vi "Get Master and Local Mod IOVs.vi"(6 "Disable Refresh Modules":bool, 8 "error in (no error)":errorcluster, 11 "IOV Engine in":refnum<k21>="ni.var.io:/") -> (0 "error IO":errorcluster, 1 "All Masters":refnum<k21>[](array[refnum]), 2 "All Local Mods":refnum<k21>[](array[refnum]), 3 "Local UDV Container":refnum<k21>[](array[refnum]))   [LabVIEW 2020, in "SEECD Engine.lvlib"]
uses:
  SEECD Engine.lvlib
  <resource>/objmgr/ni.var.rc
  <vilib>/NI VeriStand/Custom Device Tools/Custom Device Utility Library/Custom Device Utility Library.lvlib
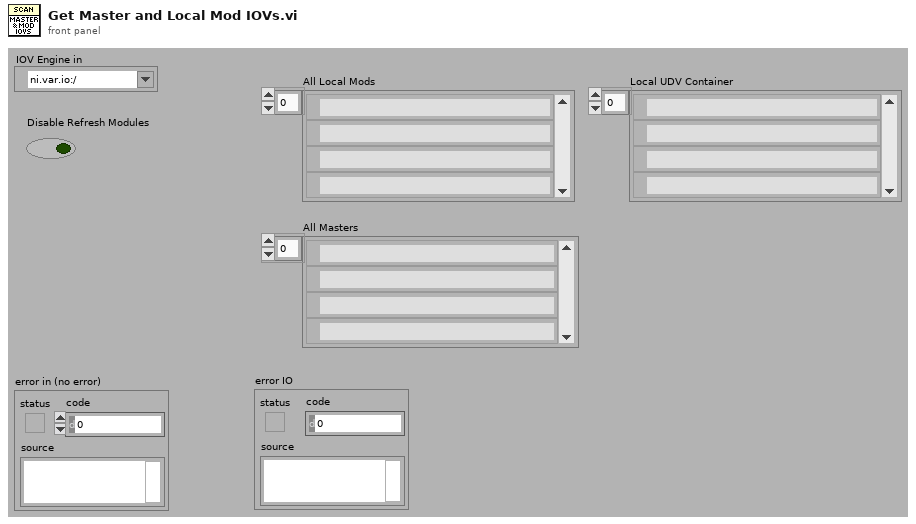
[diagram p1: front panel]
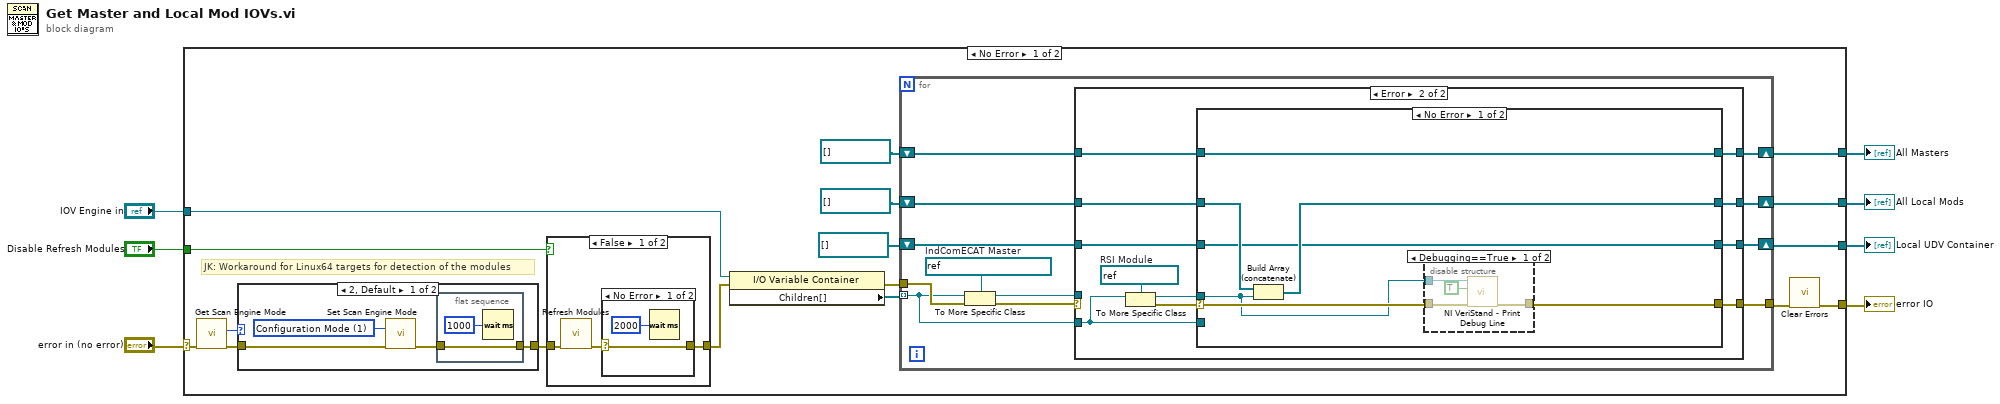
[diagram p0: block diagram]
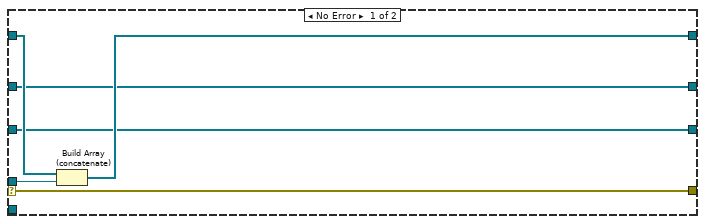
[diagram p5: hidden frame]
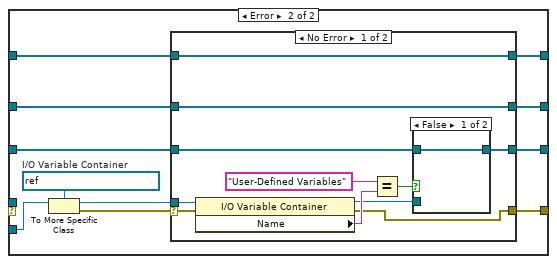
[diagram p7: hidden frame]
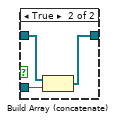
[diagram p8: hidden frame]
diagram:
  n1 = case shown="No Error" "error in (no error)" {
    selector: "error in (no error)" -> [w11 w110]
    tunnel: [w24 w110] -> w7
    tunnel: [w21 _] -> w6
    tunnel: "IOV Engine in" -> [w18 _]
    tunnel: [w16 _] -> w3
    tunnel: [w14 _] -> w2
    tunnel: "Disable Refresh Modules" -> [w8 _]
    frame No Error {
      # "JK: Workaround for Linux64 targets for detection of the modules"
      n2 = call <vilib>:"Get Scan Engine Mode.vi"("error in (no error)"=w11) -> ("error out"=w13:errorcluster, "mode"=w12:i32)  [unwired: 9 in]
      n3 = case shown="2, Default" w12 {
        tunnel: w13 -> [w34 w38]
        tunnel: [w33 w38] -> w9
        frame 2, Default {
          w35 = 1 items=["Configuration Mode"=1, "Active Mode"=2] ("mode (Active Mode)")
          n4 = call <vilib>:"Set Scan Engine Mode.vi"("mode (Active Mode)"=w35, "error in (no error)"=w34) -> ("error out"=w32:errorcluster)  [unwired: 13 in]
          n5 = flat-sequence {
            tunnel: [w37] -> w33
            tunnel: w32 -> [w37]
            frame #0 {
              n6 = Wait (ms)(milliseconds to wait=u32 1000) -> ()  [unwired: 1 out]
            }
          }
        }
        frame 1 {
        }
      }
      n7 = case shown="False" w8 {
        tunnel: [w26 w31] -> w10
        tunnel: w9 -> [w25 w31]
        frame False {
          n8 = call <vilib>:"Refresh Modules.vi"("error in (no error)"=w25) -> ("error out"=w27:errorcluster)  [unwired: 10 in]
          n9 = case shown="No Error" w27 {
            selector: w27 -> [w28 w30]
            tunnel: [w28 w30] -> w26
            frame No Error {
              n10 = Wait (ms)(milliseconds to wait=u32 2000) -> ()  [unwired: 1 out]
            }
            frame Error {
            }
          }
        }
        frame True {
        }
      }
      n11 = property class="I/O Variable Container"(reference=w18, error in=w10) -> (error out=w20:errorcluster, "Children[]"=w19:refnum<k21>[])  [unwired: 1 out]
      n12 = for {
        tunnel: w19 -> [w43] mode=indexing
        tunnel: w20 -> [w50]
        shift-right: [w46] -> w21
        shift-left: refnum<k21>[] [] -> [w45]
        tunnel: [w44] -> w23
        shift-right: [w41] -> w16
        shift-left: refnum<k21>[] [] -> [w42]
        shift-right: [w39] -> w14
        shift-left: refnum<k21>[] [] -> [w40]
        w49 = refnum<k21> refnum  # IndComECAT Master
        n13 = To More Specific Class(target class=w49, reference=w43, error in=w50) -> (specific class reference=w47:refnum<k21>, error out=w48:errorcluster)
        n14 = case shown="Error" w48 {
          selector: w48 -> [w54 _]
          tunnel: w47 -> [w51 _]
          tunnel: [w56 w61] -> w46
          tunnel: w45 -> [w55 w62]
          tunnel: [w54 w60] -> w44
          tunnel: w43 -> [_ w59]
          tunnel: w42 -> [w53 w64]
          tunnel: [w53 w63] -> w41
          tunnel: w40 -> [w52 w58]
          tunnel: [w52 w57] -> w39
          frame No Error {
            n15 = Build Array (concatenate)(w55, w51) -> (w56:refnum<k21>[])
          }
          frame Error {
            w67 = refnum<k21> refnum  # RSI Module
            n16 = To More Specific Class(target class=w67, reference=w59) -> (specific class reference=w65:refnum<k21>, error out=w66:errorcluster)  [unwired: 1 in]
            n17 = case shown="No Error" w66 {
              tunnel: w65 -> [w68 _]
              selector: w66 -> [w69 _]
              tunnel: w64 -> [w74 w86]
              tunnel: [w73 w83] -> w63
              tunnel: w62 -> [w72 w85]
              tunnel: [w72 w84] -> w61
              tunnel: [w70 w80] -> w60
              tunnel: w59 -> [_ w89]
              tunnel: w58 -> [w71 w87]
              tunnel: [w71 w82] -> w57
              frame No Error {
                n18 = Build Array (concatenate)(w74, w68) -> (w73:refnum<k21>[])
                n19 = disable-structure shown="Debugging==True" {
                  disable-tunnel: [w78 w79] -> w70
                  disable-tunnel: w69 -> [w77 w79]
                  disable-tunnel: w68 -> [w76 _]
                  frame condition #0 {
                    n20 = call <vilib>:"NI VeriStand - Print Debug Line.vi"("error in (no error)"=w77, "Add to log file? (F)"=TRUE, "Message"=w76) -> ("error out"=w78:errorcluster)  [unwired: 8 in]
                  }
                  frame condition #1 (active) {
                  }
                }
              }
              frame Error {
                w90 = refnum<k21> refnum  # I/O Variable Container
                n21 = To More Specific Class(target class=w90, reference=w89) -> (specific class reference=w81:refnum<k21>, error out=w88:errorcluster)  [unwired: 1 in]
                n22 = case shown="No Error" w88 {
                  selector: w88 -> [w99 w106]
                  tunnel: w87 -> [w93 w109]
                  tunnel: w86 -> [w100 w108]
                  tunnel: w85 -> [w101 w107]
                  tunnel: [w101 w107] -> w84
                  tunnel: [w100 w108] -> w83
                  tunnel: [w92 w109] -> w82
                  tunnel: w81 -> [w98 _]
                  tunnel: [w91 w106] -> w80
                  frame No Error {
                    n23 = property class="I/O Variable Container"(reference=w98, error in=w99) -> (reference out=w94:refnum<k21>, error out=w91:errorcluster, "Name"=w97:string)
                    n24 = Equal?(x="User-Defined Variables", y=w97) -> (x = y?=w95:bool)
                    n25 = case shown="False" w95 {
                      tunnel: w94 -> [_ w104]
                      tunnel: w93 -> [w102 w105]
                      tunnel: [w102 w103] -> w92
                      frame False {
                      }
                      frame True {
                        n26 = Build Array (concatenate)(w105, w104) -> (w103:refnum<k21>[])
                      }
                    }
                  }
                  frame Error {
                  }
                }
              }
            }
          }
        }
      }
      n27 = call <vilib>:"Clear Errors.vi"("error in (no error)"=w23) -> ("error out"=w24:errorcluster)  [unwired: 5 in, 1 out]
    }
    frame Error {
    }
  }
  "All Masters" <- w6
  "error IO" <- w7
  "All Local Mods" <- w3
  "Local UDV Container" <- w2
